vi "Handle Debug Data.vi"(7 "Action":T1(ring), 8 "error in (no error)":errorcluster, 9 "Message Data":variant, 10 "Message":string, 11 "Process In":refnum<class "Process.lvclass">) -> (0 "error out":errorcluster, 3 "Process Out":refnum<class "Process.lvclass">)   [LabVIEW 2020, in "Process.lvclass"]
doc: "Record data for debugging purposes."
uses:
  Process.lvclass
  Process.lvclass/Process.ctl
  Logging/Logging.lvclass
  C:/git/astemes-triarc-framework/source/Framework/Base/Base.lvclass
  C:/git/astemes-triarc-framework/source/Framework/Process/Process.lvclass
  C:/git/astemes-triarc-framework/source/Framework/Error Handler Interface/Error Handler Interface.lvclass
  C:/git/astemes-triarc-framework/source/Framework/Logging/Logging.lvclass
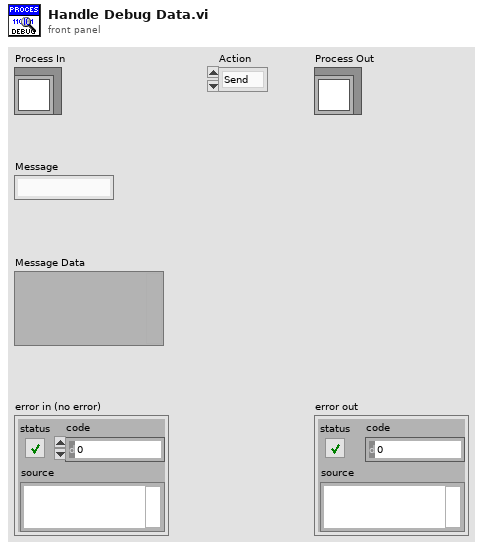
[diagram p1: front panel]
types:
  T1 = enum16{"Send", "Receive", "Request", "Response", "Broadcast"}
  T2 = cluster{"Action":string, "Call Chain":string, "Process":string, "Message":string, "Message Data":variant, "Time":dbl}
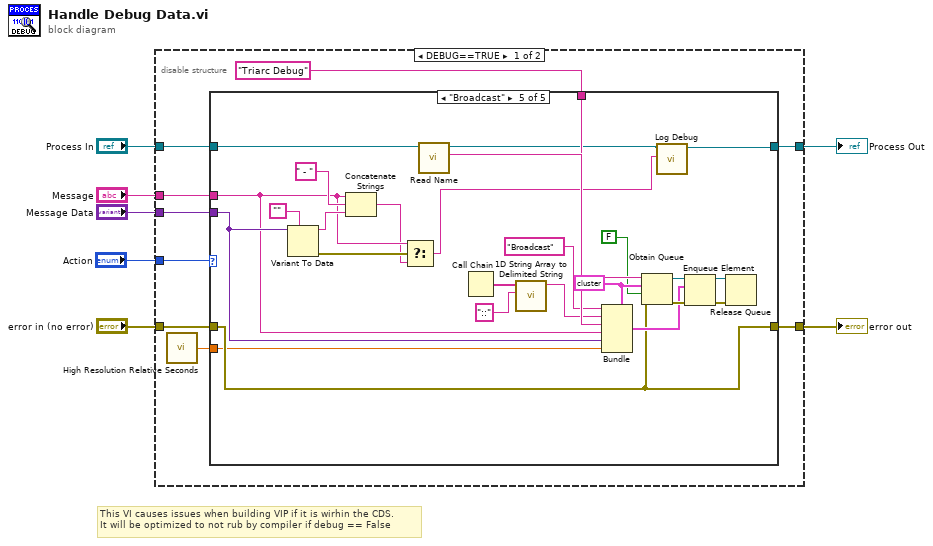
[diagram p0: block diagram]
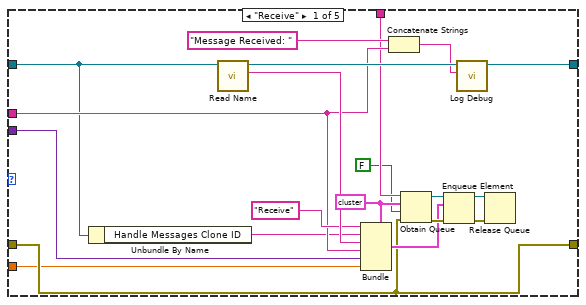
[diagram p2: hidden frame]
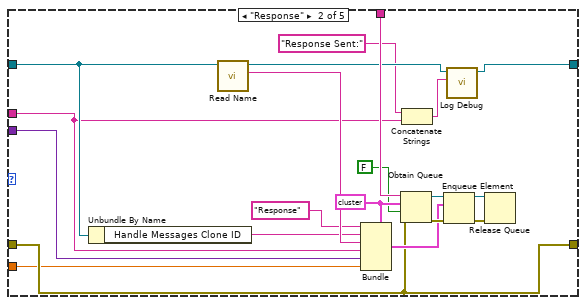
[diagram p3: hidden frame]
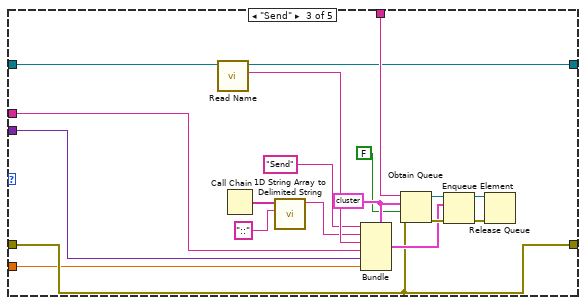
[diagram p4: hidden frame]
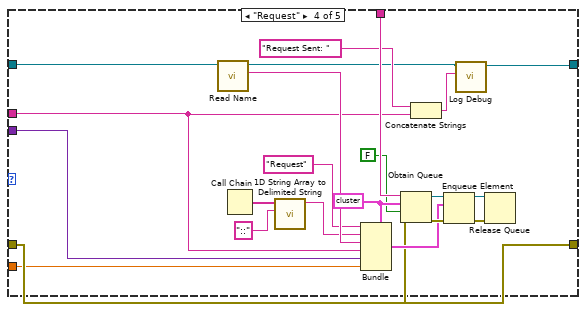
[diagram p5: hidden frame]
diagram:
  # "This VI causes issues when building VIP if it is wirhin the CDS.\nIt will be optimized to not rub by compiler if debug == False"
  n1 = disable-structure shown="DEBUG==TRUE" {
    disable-tunnel: "Message" -> [w14 _]
    disable-tunnel: "Message Data" -> [w16 _]
    disable-tunnel: [w15 w125] -> w4
    disable-tunnel: "Process In" -> [w13 w125]
    disable-tunnel: [w12 w124] -> w5
    disable-tunnel: "error in (no error)" -> [w11 w124]
    disable-tunnel: "Action" -> [w10 _]
    frame condition #0 (active) {
      n2 = call <vilib>:"High Resolution Relative Seconds.vi"() -> ("relative seconds"=w8:dbl)
      n3 = case shown="\"Broadcast\"" w10 {
        tunnel: w16 -> [w28 w48 w65 w87 w102]
        tunnel: [w26 w39 w58 w77 w106] -> w15
        tunnel: w14 -> [w23 w37 w57 w76 w100]
        tunnel: w13 -> [w22 w47 w64 w86 w113]
        tunnel: [w18 w43 w60 w83 w110] -> w12
        tunnel: w11 -> [w18 w43 w60 w83 w110]
        tunnel: "Triarc Debug" ("name (unnamed)") -> [w20 w45 w62 w84 w111]
        tunnel: w8 -> [w17 w42 w59 w81 w108]
        frame "Receive" {
          w35 = T2 {"Action"="", "Call Chain"="", "Process"="", "Message"="", "Message Data"=variant, "Time"=0.0} ("output cluster")
          n4 = Unbundle By Name(w22) -> ("Handle Messages Clone ID"=w21:string)
          n5 = call "Read Name.vi"("Process In"=w22) -> ("Qualified Name"=w36:string, "Process Out"=w27:refnum<class "Process.lvclass">)  [unwired: 7 in, 2 out]
          n6 = Bundle(cluster=w35, "Action"="Receive", "Call Chain"=w21, "Process"=w36, "Message"=w23, "Message Data"=w28, "Time"=w17) -> (w32:T2)
          n7 = Concatenate Strings("Message Received: " ("name (unnamed)"), w23) -> (w24:string)
          n8 = Obtain Queue(name (unnamed)=w20, element data type=w35, create if not found? (T)=FALSE, error in (no error)=w18) -> (queue out=w34:refnum<queue>, error out=w33:errorcluster)  [unwired: 1 in, 1 out]
          n9 = Enqueue Element(queue=w34, element=w32, error in (no error)=w33) -> (queue out=w31:refnum<queue>, error out=w30:errorcluster)  [unwired: 1 in, 1 out]
          n10 = call "Log Debug.vi"("Message"=w24, "Logging In"=w27) -> ("Logging Out"=w26:refnum<class "Process.lvclass">)  [unwired: 8 in, 1 out]
          n11 = Release Queue(queue=w31, error in (no error)=w30) -> ()  [unwired: 1 in, 3 out]
        }
        frame "Response" {
          w55 = T2 {"Action"="", "Call Chain"="", "Process"="", "Message"="", "Message Data"=variant, "Time"=0.0} ("output cluster")
          n12 = Unbundle By Name(w47) -> ("Handle Messages Clone ID"=w46:string)
          n13 = call "Read Name.vi"("Process In"=w47) -> ("Qualified Name"=w56:string, "Process Out"=w40:refnum<class "Process.lvclass">)  [unwired: 7 in, 2 out]
          n14 = Bundle(cluster=w55, "Action"="Response", "Call Chain"=w46, "Process"=w56, "Message"=w37, "Message Data"=w48, "Time"=w42) -> (w52:T2)
          n15 = Obtain Queue(name (unnamed)=w45, element data type=w55, create if not found? (T)=FALSE, error in (no error)=w43) -> (queue out=w54:refnum<queue>, error out=w53:errorcluster)  [unwired: 1 in, 1 out]
          n16 = Concatenate Strings("Response Sent:", w37) -> (w41:string)
          n17 = Enqueue Element(queue=w54, element=w52, error in (no error)=w53) -> (queue out=w51:refnum<queue>, error out=w50:errorcluster)  [unwired: 1 in, 1 out]
          n18 = call "Log Debug.vi"("Message"=w41, "Logging In"=w40) -> ("Logging Out"=w39:refnum<class "Process.lvclass">)  [unwired: 8 in, 1 out]
          n19 = Release Queue(queue=w51, error in (no error)=w50) -> ()  [unwired: 1 in, 3 out]
        }
        frame "Send" {
          w63 = T2 {"Action"="", "Call Chain"="", "Process"="", "Message"="", "Message Data"=variant, "Time"=0.0} ("output cluster")
          n20 = call "Read Name.vi"("Process In"=w64) -> ("Qualified Name"=w75:string, "Process Out"=w58:refnum<class "Process.lvclass">)  [unwired: 7 in, 2 out]
          n21 = Call Chain() -> (call chain=w74:string[])
          n22 = call <vilib>:"1D String Array to Delimited String.vi"("delimiter"="::", "string array"=w74) -> ("delimited string"=w72:string)  [unwired: 9 in]
          n23 = Bundle(cluster=w63, "Action"="Send", "Call Chain"=w72, "Process"=w75, "Message"=w57, "Message Data"=w65, "Time"=w59) -> (w69:T2)
          n24 = Obtain Queue(name (unnamed)=w62, element data type=w63, create if not found? (T)=FALSE, error in (no error)=w60) -> (queue out=w71:refnum<queue>, error out=w70:errorcluster)  [unwired: 1 in, 1 out]
          n25 = Enqueue Element(queue=w71, element=w69, error in (no error)=w70) -> (queue out=w68:refnum<queue>, error out=w67:errorcluster)  [unwired: 1 in, 1 out]
          n26 = Release Queue(queue=w68, error in (no error)=w67) -> ()  [unwired: 1 in, 3 out]
        }
        frame "Request" {
          w85 = T2 {"Action"="", "Call Chain"="", "Process"="", "Message"="", "Message Data"=variant, "Time"=0.0} ("output cluster")
          n27 = call "Read Name.vi"("Process In"=w86) -> ("Qualified Name"=w97:string, "Process Out"=w78:refnum<class "Process.lvclass">)  [unwired: 7 in, 2 out]
          n28 = Call Chain() -> (call chain=w96:string[])
          n29 = call <vilib>:"1D String Array to Delimited String.vi"("delimiter"="::", "string array"=w96) -> ("delimited string"=w94:string)  [unwired: 9 in]
          n30 = Bundle(cluster=w85, "Action"="Request", "Call Chain"=w94, "Process"=w97, "Message"=w76, "Message Data"=w87, "Time"=w81) -> (w91:T2)
          n31 = Obtain Queue(name (unnamed)=w84, element data type=w85, create if not found? (T)=FALSE, error in (no error)=w83) -> (queue out=w93:refnum<queue>, error out=w92:errorcluster)  [unwired: 1 in, 1 out]
          n32 = Concatenate Strings("Request Sent: " ("name (unnamed)"), w76) -> (w80:string)
          n33 = Enqueue Element(queue=w93, element=w91, error in (no error)=w92) -> (queue out=w90:refnum<queue>, error out=w89:errorcluster)  [unwired: 1 in, 1 out]
          n34 = call "Log Debug.vi"("Message"=w80, "Logging In"=w78) -> ("Logging Out"=w77:refnum<class "Process.lvclass">)  [unwired: 8 in, 1 out]
          n35 = Release Queue(queue=w90, error in (no error)=w89) -> ()  [unwired: 1 in, 3 out]
        }
        frame "Broadcast" {
          w112 = T2 {"Action"="", "Call Chain"="", "Process"="", "Message"="", "Message Data"=variant, "Time"=0.0} ("output cluster")
          n36 = Variant To Data(type="", Variant=w102) -> (data=w103:string, error out=w101:errorcluster)  [unwired: 1 in]
          n37 = Concatenate Strings(w100, " - " ("string"), w103) -> (w99:string)
          n38 = Select(t=w100, s=w101, f=w99) -> (s? t:f=w98:string)
          n39 = call "Read Name.vi"("Process In"=w113) -> ("Qualified Name"=w123:string, "Process Out"=w107:refnum<class "Process.lvclass">)  [unwired: 7 in, 2 out]
          n40 = Call Chain() -> (call chain=w122:string[])
          n41 = call <vilib>:"1D String Array to Delimited String.vi"("delimiter"="::", "string array"=w122) -> ("delimited string"=w120:string)  [unwired: 9 in]
          n42 = Bundle(cluster=w112, "Action"="Broadcast", "Call Chain"=w120, "Process"=w123, "Message"=w100, "Message Data"=w102, "Time"=w108) -> (w117:T2)
          n43 = Obtain Queue(name (unnamed)=w111, element data type=w112, create if not found? (T)=FALSE, error in (no error)=w110) -> (queue out=w119:refnum<queue>, error out=w118:errorcluster)  [unwired: 1 in, 1 out]
          n44 = call "Log Debug.vi"("Message"=w98, "Logging In"=w107) -> ("Logging Out"=w106:refnum<class "Process.lvclass">)  [unwired: 8 in, 1 out]
          n45 = Enqueue Element(queue=w119, element=w117, error in (no error)=w118) -> (queue out=w116:refnum<queue>, error out=w115:errorcluster)  [unwired: 1 in, 1 out]
          n46 = Release Queue(queue=w116, error in (no error)=w115) -> ()  [unwired: 1 in, 3 out]
        }
      }
    }
    frame condition #1 {
    }
  }
  "error out" <- w5
  "Process Out" <- w4
